vi "产品侧.vi"() -> ()   [LabVIEW 2026]
doc: "产品运转测控界面 - APS 设备侧计量 主页面（命令与模拟量）。仅前面板布局演示，无程序逻辑。来源：产品侧.html 主界面。"
panel:
  out "53 状态栏-版本":string="APS 测控系统 V2.0"
  out "52 状态栏-帧计数":string="帧计数: 0000 | 采样周期: 20 ms | 通道数: 128"
  out "51 状态栏-通讯":string="● 通讯正常 | ● 采集运行中"
  out "50 APU排气温度趋势":waveform(dbl)(graph)
  in  "模拟量·滑油温度(℃)":dbl
  in  "模拟量·进气门位置(°)":dbl
  in  "模拟量·燃油压力(kPa)":dbl=210.0
  in  "模拟量·主燃油伺服电流(mA)":dbl
  in  "模拟量·功率输出电流(A)":dbl
  in  "模拟量·APSC供电电压(V)":dbl
  in  "模拟量·气瓶温度(℃)":dbl
  in  "模拟量·气瓶压力(MPa)":dbl
  in  "模拟量·俯仰角(°)":dbl
  in  "模拟量·校准空速(km/h)":dbl
  in  "模拟量·马赫数":dbl
  in  "模拟量·气压高度(m)":dbl
  in  "模拟量·右发转速(%)":dbl
  in  "模拟量·左发转速(%)":dbl
  out "49 有效位·大气总温数据有效":bool=TRUE
  out "48 有效位·马赫数数据有效":bool
  out "47 有效位·燃油温度有效位1":bool
  out "46 有效位·气压高度数据有效":bool=TRUE
  out "45 有效位·燃油温度有效位0":bool
  out "44 有效位·发动机高压转子转速有效":bool=TRUE
  out "43 仪表·供电电压(V)":dbl=28.2
  out "42 仪表·燃油压力(kPa)":dbl=210.0
  out "41 仪表·引气温度(℃)":dbl=128.0
  out "40 仪表·滑油压力(kPa)":dbl=315.0
  out "39 仪表·排气温度(℃)":dbl=486.0
  out "38 仪表·APU转速(%)":dbl=72.0
  out "37 系统信号流":string="RIU (命令/模拟量) → APSC (辅助动力控制器) → APU (辅助动力装置) → ATS (引气关断阀)"
  in  "在线加载状态":i32(ring) items=["正常工作模式", "维护模式", "加载模式"]
  in  "校验和":i32
  in  "数据长度":i32
  in  "数据包标识":i32
  in  "帧计数":i32
  out "36 APSC发送报文":string="AA55 0040 0000 0000 0000 0000 0000 0000 0000 0000 FFF0 0100 0000 0000 0000 0000 0000 0000 0000 0000 0000 0000 4E64"
  out "35 状态字·正常工作模式":bool=TRUE
  out "34 状态字·电源系统请求起动辅助动力":bool
  out "33 状态字·右发假起动":bool
  out "32 状态字·左发假起动":bool
  out "31 状态字·地面":bool
  out "30 通讯故障·预留2":bool
  out "29 通讯故障·预留1":bool
  out "28 通讯故障·发送数据失效":bool
  out "27 通讯故障·发送RIU2B数据故障":bool
  out "26 通讯故障·发送RIU1C数据故障":bool
  out "25 命令字·关闭进排气门":bool
  out "24 命令字·打开进排气门":bool
  out "23 命令字·停止系统维护":bool
  out "22 命令字·空气能源系统气瓶放气":bool
  out "21 命令字·EPU气密性检查":bool
  out "20 命令字·EPU管路排气":bool
  out "19 命令字·EPU油瓶放油":bool
  out "18 命令字·EPU油瓶手动加油":bool
  out "17 命令字·EPU冷运转":bool
  out "16 命令字·85%磨合(地面测试设备用)":bool
  out "15 命令字·70%磨合(地面测试设备用)":bool
  out "14 命令字·50%磨合(地面测试设备用)":bool
  out "13 命令字·APU假起动":bool
  out "12 命令字·APU冷运转":bool
  out "11 命令字·GMP停机APU":bool
  out "10 命令字·GMP启动APU":bool
  out "09 命令字·环控使用APU引气需求":bool
  out "08 命令字·打开右ATS引气关断阀":bool
  out "07 命令字·打开左ATS引气关断阀":bool
  out "06 命令字·辅助动力自动停车":bool
  out "05 命令字·辅助动力自动起动请求":bool
  in  "命令字·读取APSC系统及关键LRU":bool
  in  "命令字·系统运行命令":bool=TRUE
  in  "开关·关闭进排气门":bool
  in  "开关·打开进排气门":bool=TRUE
  in  "开关·GMP停机APU":bool
  in  "开关·GMP启动APU":bool
  in  "开关·环控使用APU引气需求":bool=TRUE
  in  "开关·打开右ATS引气关断阀":bool
  in  "开关·打开左ATS引气关断阀":bool=TRUE
  in  "开关·APU假起动":bool=TRUE
  in  "开关·APU冷运转":bool
  in  "开关·辅助动力自动停车":bool
  in  "开关·辅助动力自动起动请求":bool=TRUE
  in  "开关·系统运行命令":bool=TRUE
  out "04 联机灯":bool
  out "03 系统就绪灯":bool=TRUE
  out "02 时钟":string="00:00:00"
  out "01 标题栏":string="产品运转测控"
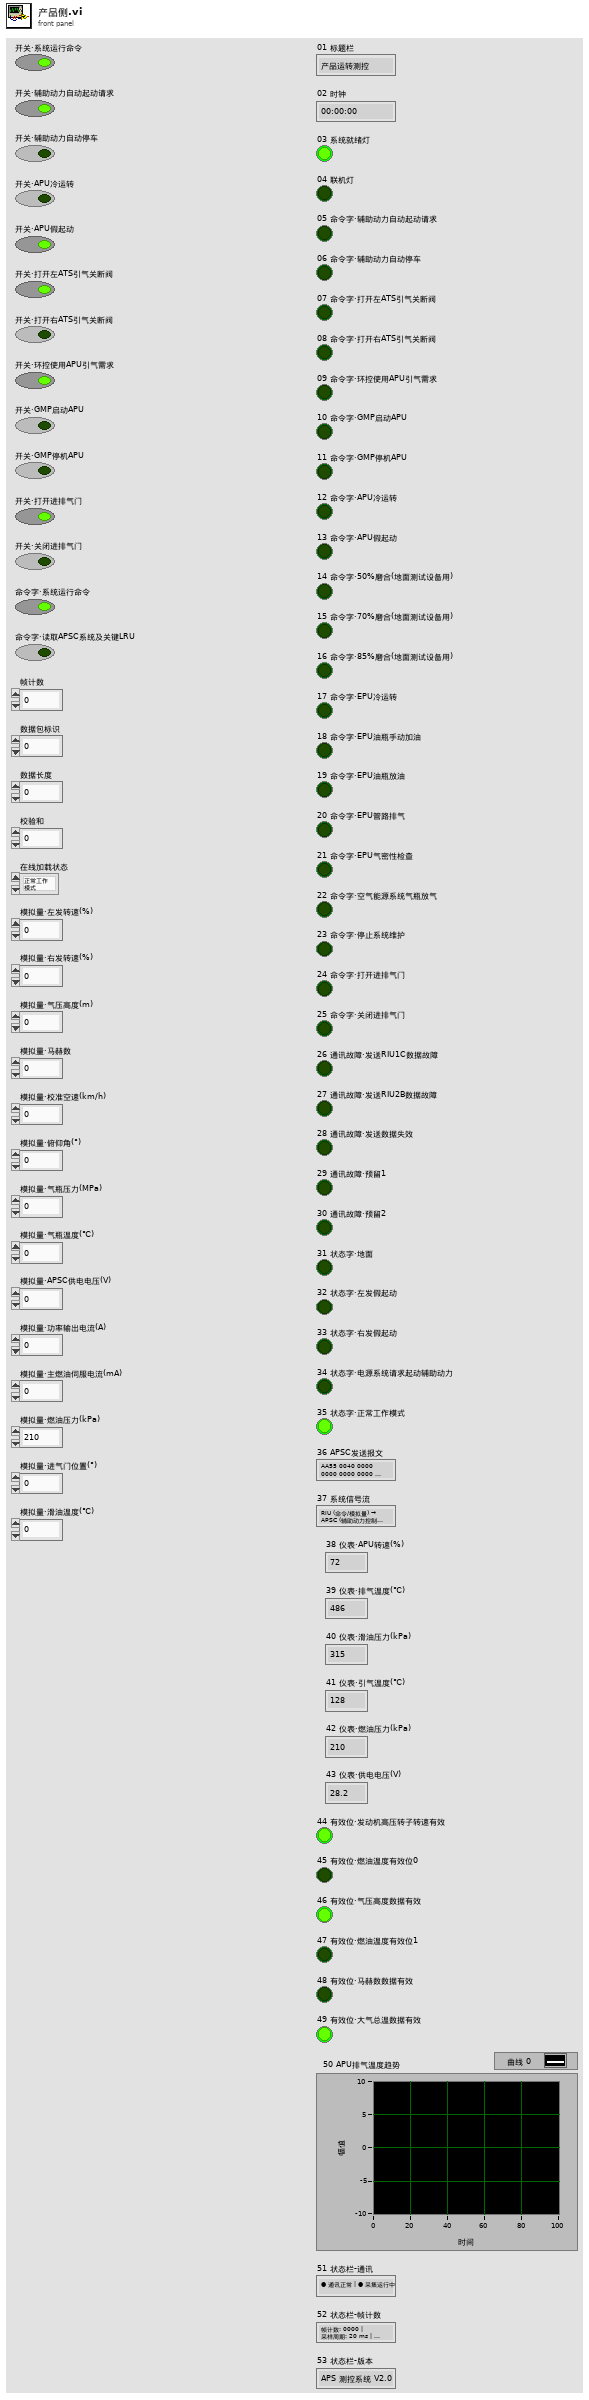
[diagram p1: front panel]
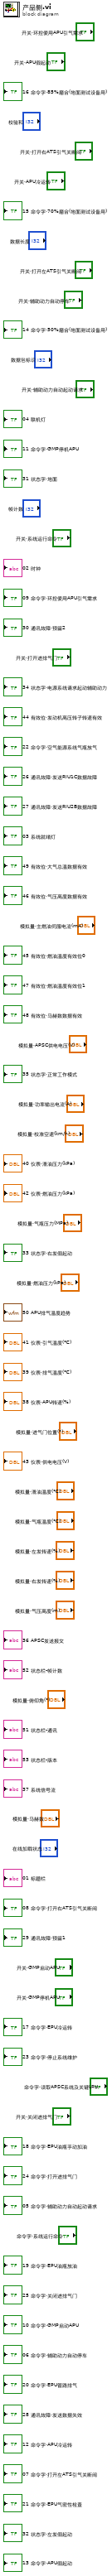
[diagram p0: block diagram]
diagram:
